vi "jymove.vi"() -> ()   [LabVIEW 2021]
uses:
  <vilib>/Math Plots/3D Math Plots/3D Scatter/3D Scatter XCtrl/3D Scatter.xctl
  <vilib>/Utility/file.llb/Write Delimited Spreadsheet (DBL).vi
  <vilib>/Math Plots/3D Math Plots/3D Scatter/3D Scatter Datatype/Public/Plot Helper (Matrix).vi
  <vilib>/Math Plots/3D Math Plots/3D Scatter/3D Scatter Datatype/3D Scatter Datatype.lvclass
  <vilib>/Analysis/NI_AALBase.lvlib
panel:
  out "Spectrum":cluster{"Y":dbl[], "Y":dbl[]}[](graph)
  out "波长数组 2":dbl[](array[numeric])
  out "data 2":i32[][](graph)
  out "Backlight":i32[][](graph)
  in  "选项卡控件":enum32{"IHR 550", "CCD", "MOVE"}(tab)
  out "Current UniqueID":string="Mono4"
  in  "Mono ID":string(combo)="Mono1"
  in  "Connect":bool
  out "Initialized JY":bool=TRUE
  in  "Force\nInitialization":bool
  in  "Target Grating":string(combo)="2"
  out "Current Description":string="1" caption="Description"
  out "Grating Index":i32=1
  out "Current Grating":dbl=1200.0
  out "Units":string="nm"
  out "Current WL":dbl=897.9988
  out "Exit Mirror\nPosition":i32(ring)=2 items=["EntranceMirror", "ExitMirror", "Front", "Side"]
  out "Entrance Mirror\nPosition":i32(ring)=2 items=["EntranceMirror", "ExitMirror", "Front", "Side"]
  out "Units 2":string="mm"
  out "Front Entrance":dbl
  in  "Target WL":dbl=710.0
  in  "Exit Mirror":u16(ring)=3 caption="Target Position Exit Mirror" items=["Front"=2, "Side"=3]
  in  "Entrance Mirror":u16(ring)=2 caption="Target Position\nEntrance Mirror" items=["Front"=2, "Side"=3]
  in  "Target\nFront Entrance":dbl=1.0
  in  "Move To\nTarget Positions":bool
  in  "initialize":bool
  in  "ShutterOpen":bool=TRUE caption="Shutter enable"
  in  "Acquire":bool
  in  "Temperature":bool
  in  "Setup":bool
  out "indicator":string="Ready !"
  in  "CCD Busy":bool
  in  "Continuous":bool
  out "initialized ?":bool=TRUE
  in  "Commande tab":T1(tab)
  in  "Area Number to Display":i32
  in  "Reformat":bool
  in  "GAIN":u16(ring)=2 caption="Device Name"
  in  "ADC":u16(ring) caption="Device Name"
  in  "Number of Areas :":u16=1 min=1 step=1
  in  "Integration time (ms) :":i16=2000
  out "Uniques ID":u16(ring)
  in  "Device Name":u16(ring)
  in  "Signal type :":enum16{"TTL Rising Edge", "TTL Falling Edge"}(ring)=enum."TTL Falling Edge"
  in  "Trigger Type :":u16(ring) items=["On Start"=1, "Per Acquisition"=2]
  in  "trigSigTypeString":string
  in  "trigEventString":string
  in  "Enable InputTriggers :":bool
  in  "Number of Cleans":i32=1
  in  "MultiAcqShutterMode":i32(ring)=3 items=["Open For All Spectra"=1, "Open for Each Spectrum"=3]
  in  "Accumulations:":u16=10 min=1 step=1
  in  "Multi Accumulation mode:":bool
  out "Y Pixels:":i32=256
  out "DataSize":i32=1024
  out "X Pixels:":i32=1024
  out "Firmware\nVersion":string="V1.20 CCD_4000"
  in  "Save Backlight":bool
  in  "起始波长":dbl=693.352
  in  "终止波长":dbl=726.407
  in  "扫描方式":enum32{"起始扫描", "半径扫描"}(tab)
  in  "y轴起始位置":sgl=5.355 min=-150 max=150 format="%#.6g"
  in  "y轴步进长度":sgl=0.0008 min=-150 max=150 format="%.4g"
  in  "y轴终止位置":sgl=5.359 min=-150 max=150 format="%#.6g"
  in  "x轴起始位置":dbl=5.495
  in  "x轴步进长度":dbl=0.0008
  in  "x轴终止位置":dbl=5.535
  in  "中心X":dbl=10.0
  in  "中心Y":dbl=10.0
  in  "X步长":dbl=0.5
  in  "Y半径":dbl=5.0
  in  "X半径":dbl=5.0
  in  "Y步长":dbl=0.5
  in  "x 位置":dbl=5.495
  in  "y 位置":sgl=5.35 min=-150 max=150 format="%#.6g"
  in  "移动":bool
  out "Acq Time(ms)":u32=3401
  out "位置":dbl[](array[numeric]) format="%.10e"
  in  "开始采集":bool
  out "采集进度":u8(slide) scale=0.0..100.0
  out "最终存储路径":path
  out "Intensity":dbl
  out "POINT":dbl
  out "JYCCDLib.IJYCCDReqd":refnum<k7>
  in  "计数器":dbl=720.0
  out "error out":errorcluster
  out "Gratings":dbl[](array[numeric])=[1200.0, 300.0]
  out "Data":i32[][](graph)
  out "trigAddress":i32
  out "Gain Number":i32[](array[numeric])=[10, 11, 12, 13, 8, 2]
  out "ADC Number":i32[](array[numeric])=[0, 1, 2, 3, 4]
  out "temp graph":dbl(graph)=-134.538067
  in  "Close":bool=TRUE
  out "areas :":i32[][](array[numeric])=[[1], [1], [1], [1024], [256], [1], [256]]
  in  "Constante de condition\n(Voir l'aide contextuelle)":bool
  out "波长3维图":refnum<class "3D Plot Datatype.lvclass">[](xcontrol)
  out "强度三维图":refnum<class "3D Plot Datatype.lvclass">[](xcontrol)
  out "起始位置":dbl[](array[numeric])
  in  "x":dbl=10.0
  in  "y":sgl=1.0 min=-150 max=150 format="%#.6g"
  out "强度数组":dbl[][](array[numeric])
  out "波长数组":dbl[][](array[numeric])
  out "X循环次数":dbl
  out "Y循环次数":sgl
  in  "Y移动量":dbl[](array[numeric]) format="%.6f"
  in  "X移动量":dbl[](array[numeric]) format="%.6f"
  in  "Group Name (250 c max)":string="XY"
  in  "PASSWORD":string="Administrator"
  in  "USER NAME":string="Administrator"
  in  "IP Address":string="192.168.0.254"
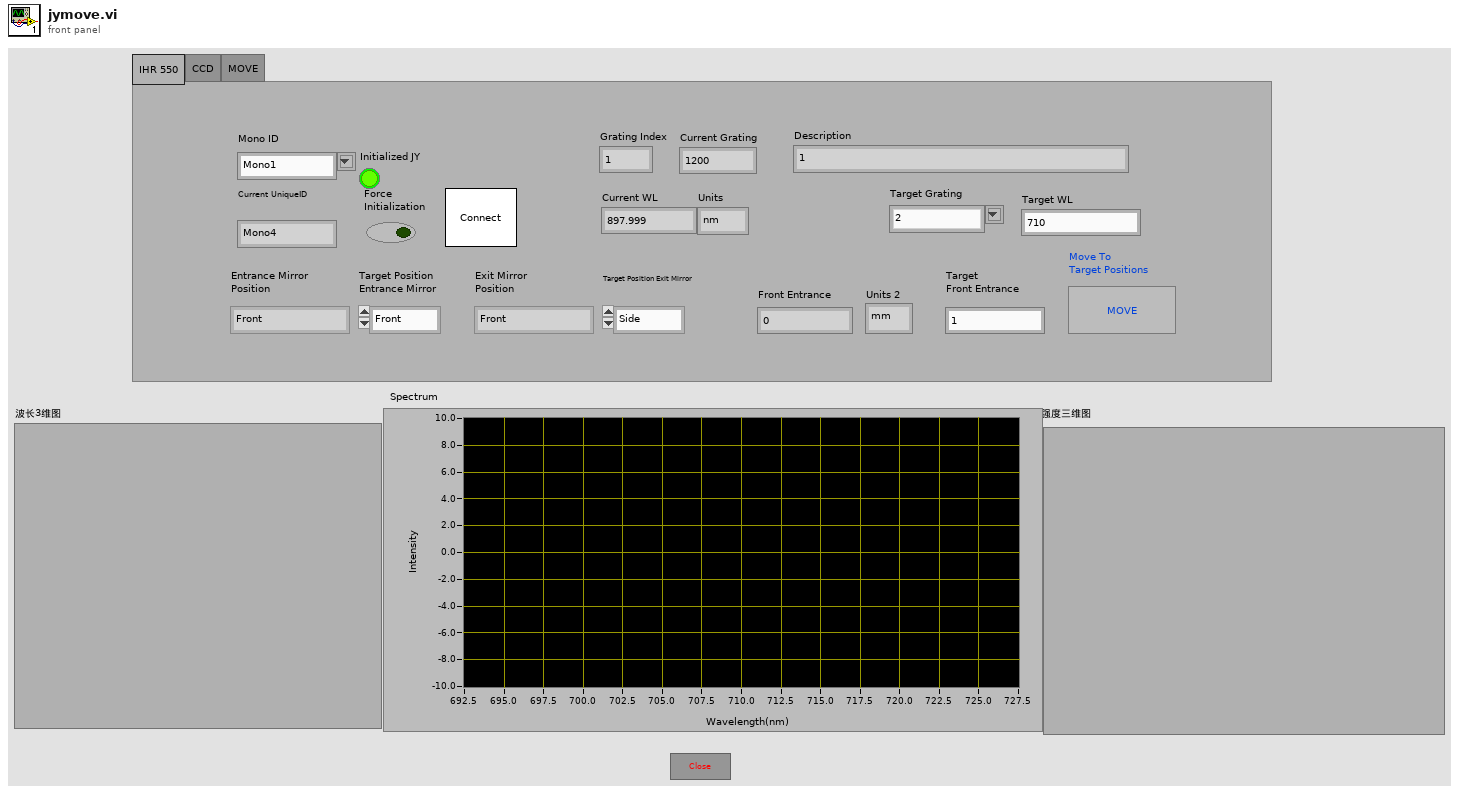
[diagram p1: front panel]
types:
  T1 = enum32{"Settings", "Trigger In", "Multi-Accu.", "Infos"}
  T2 = cluster{"connection TCP":refnum<k5>, "LogTo File":bool, "Log File refnum":refnum<file>, "no error if error log":bool}
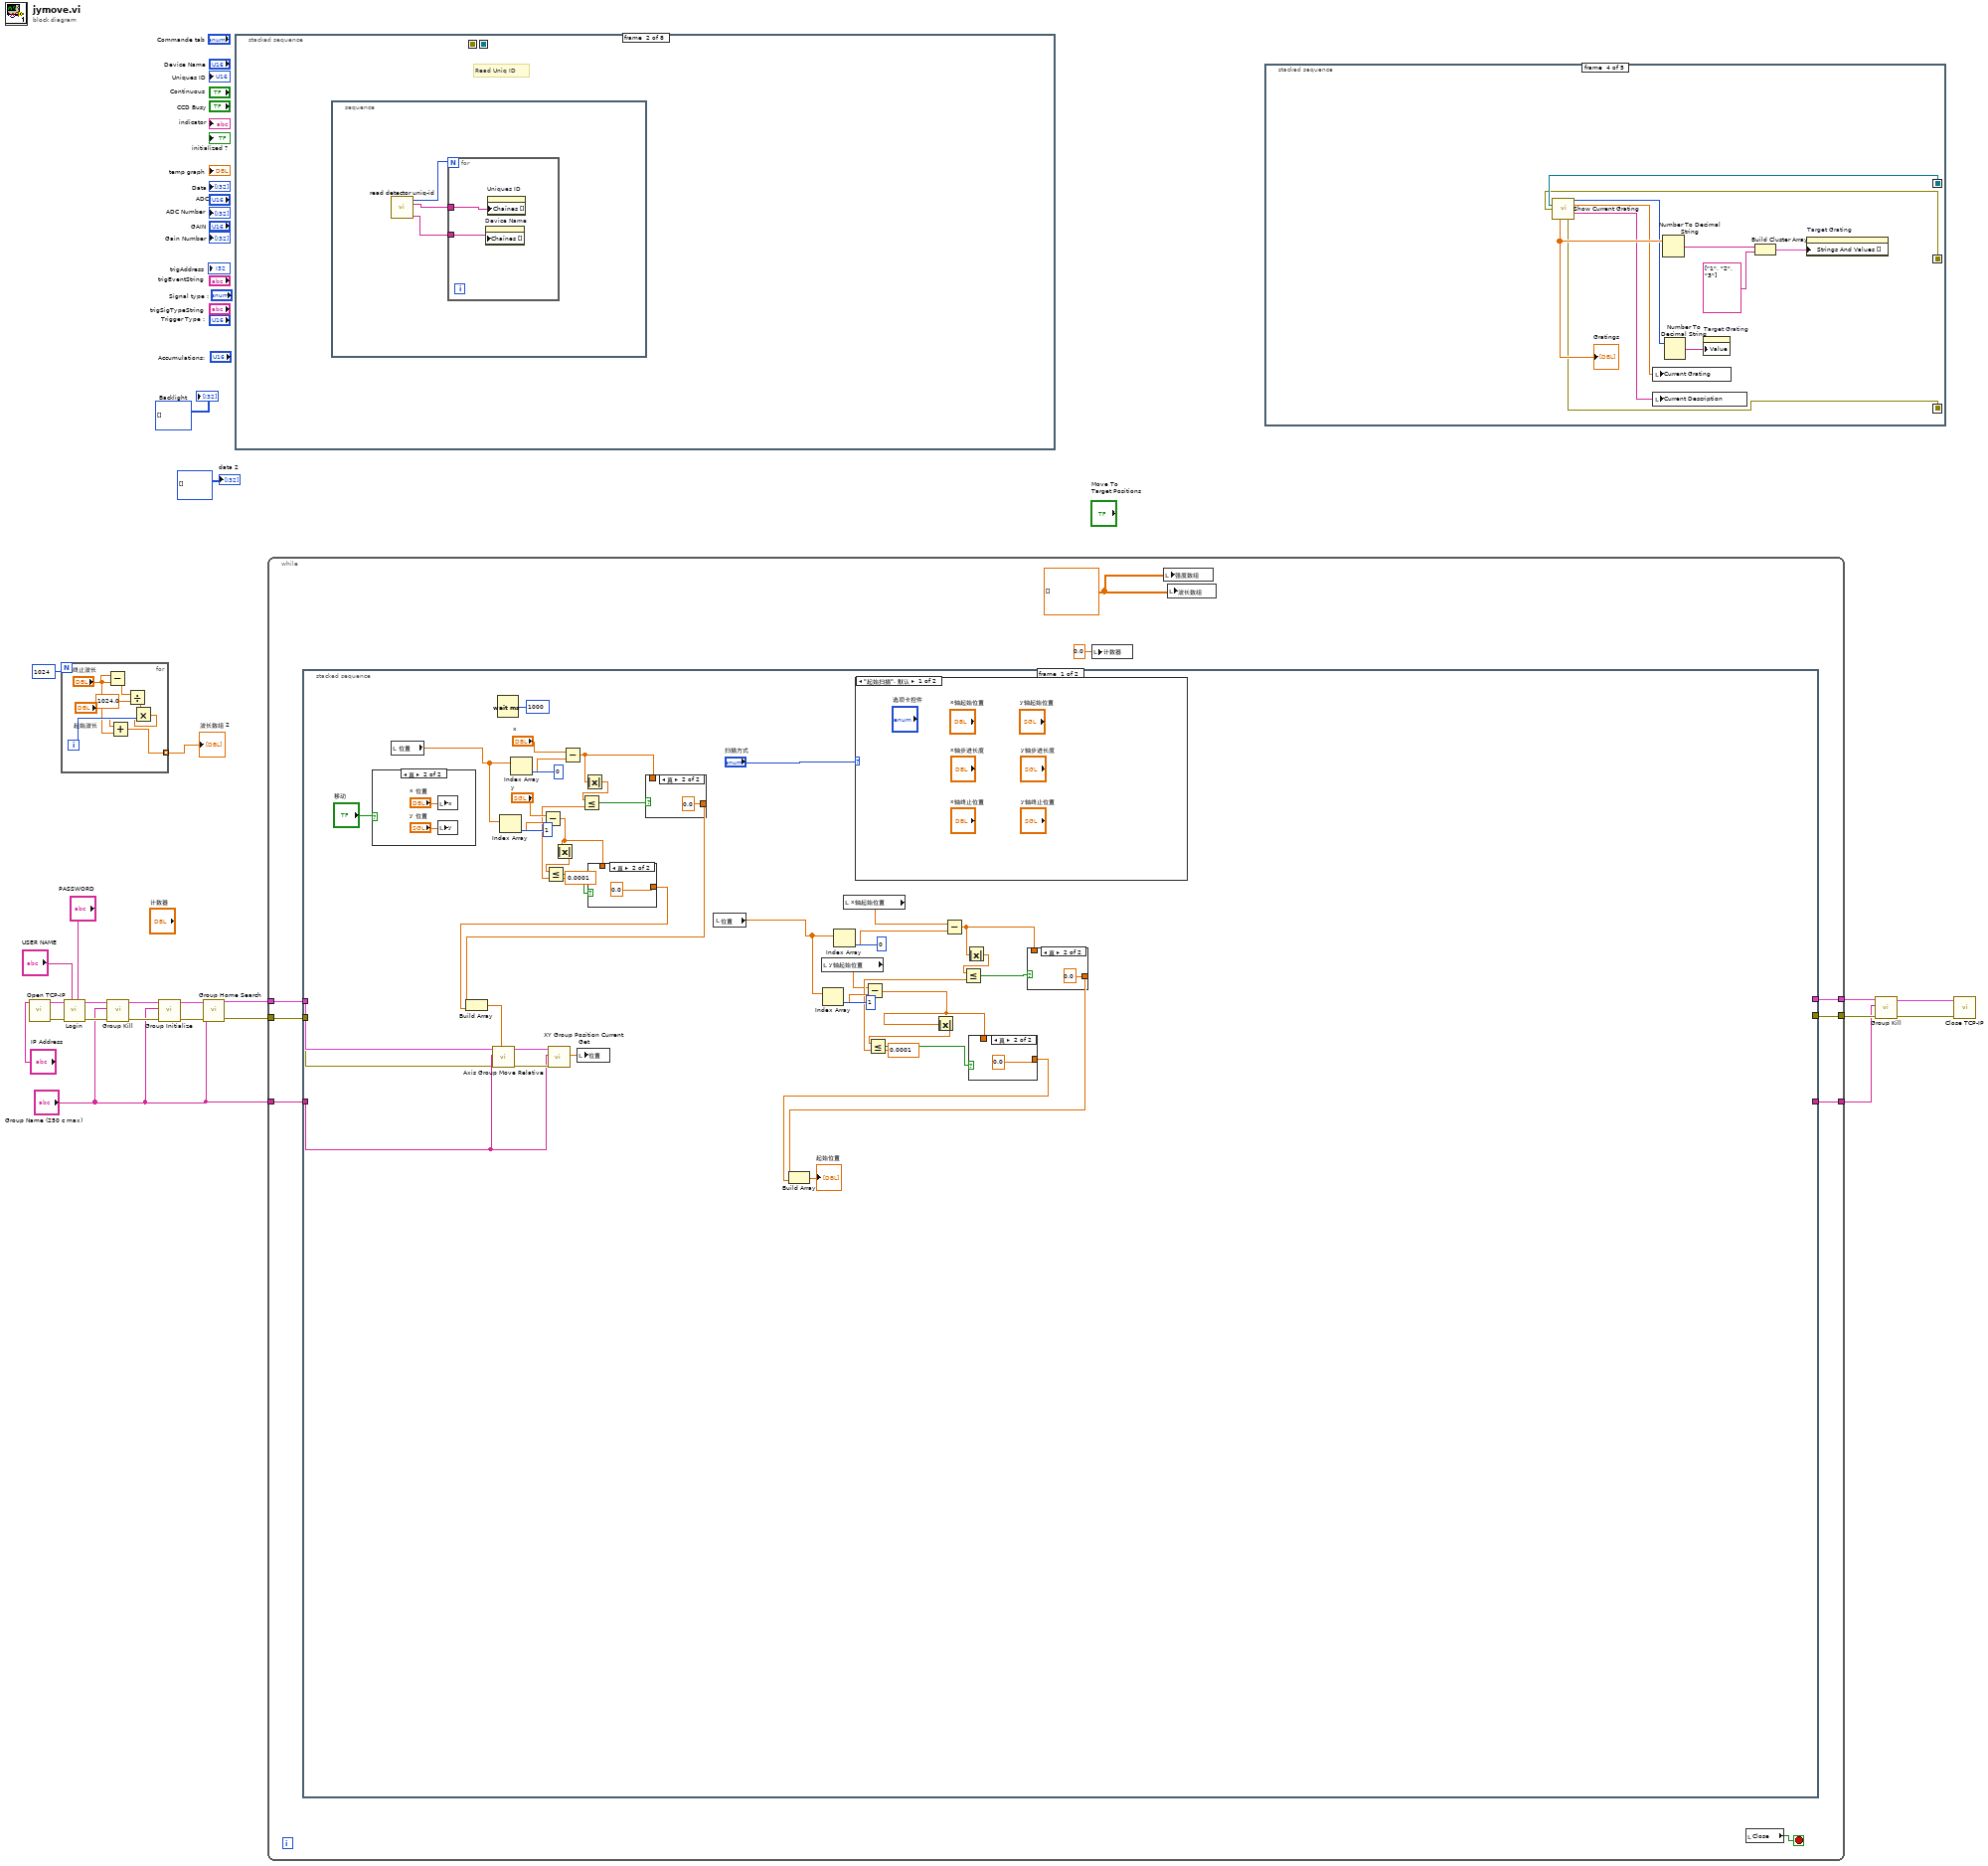
[diagram p0: block diagram]
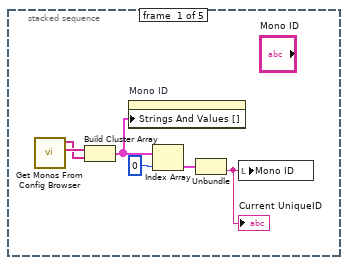
[diagram p2: hidden frame]
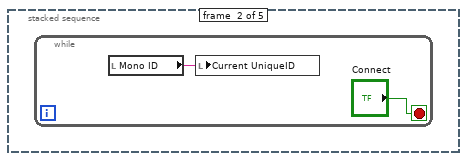
[diagram p3: hidden frame]
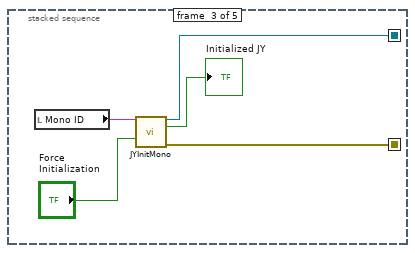
[diagram p4: hidden frame]
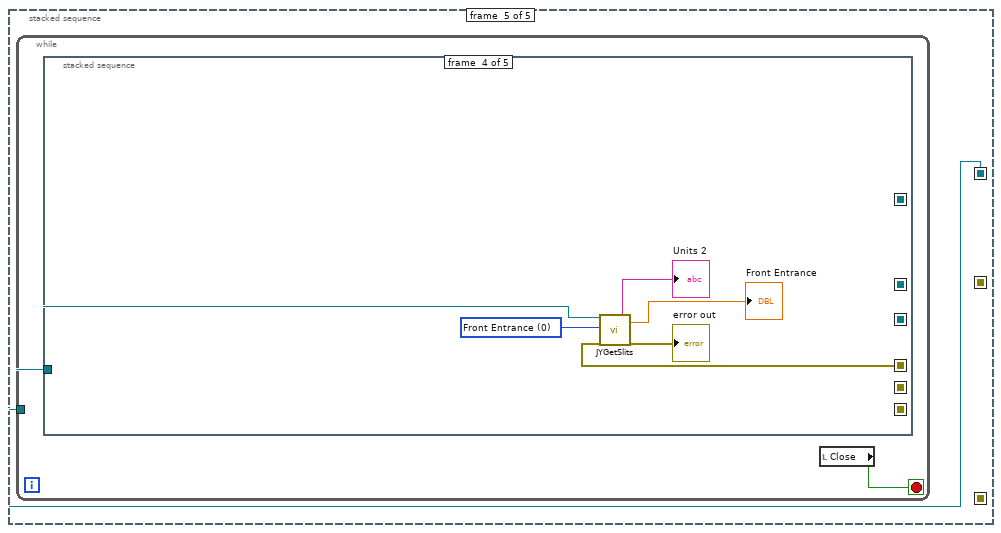
[diagram p5: hidden frame]
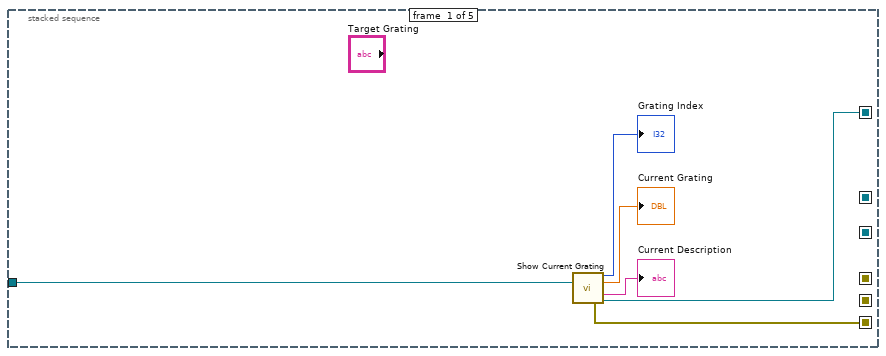
[diagram p6: hidden frame]
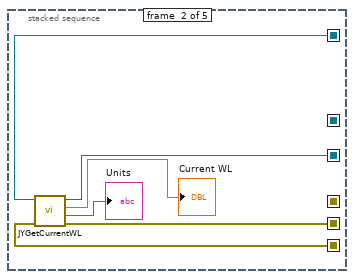
[diagram p7: hidden frame]
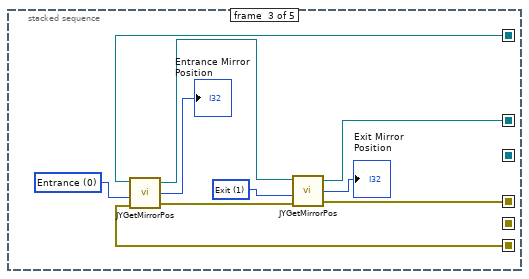
[diagram p8: hidden frame]
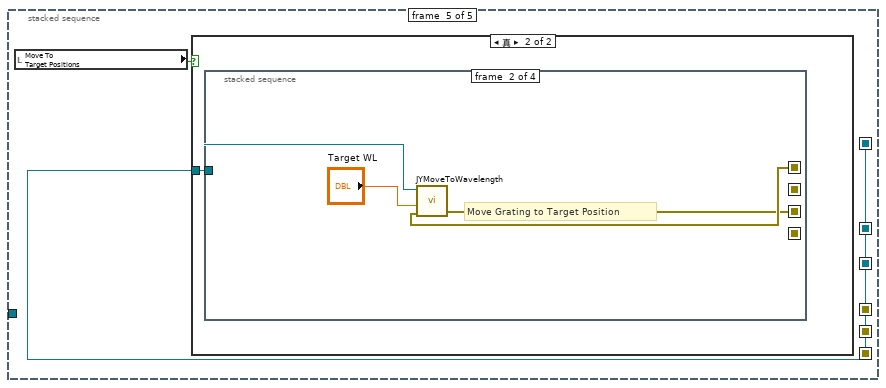
[diagram p9: hidden frame]
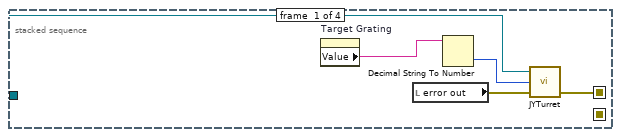
[diagram p11: hidden frame]
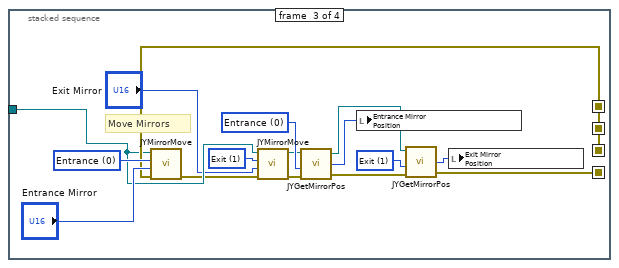
[diagram p12: hidden frame]
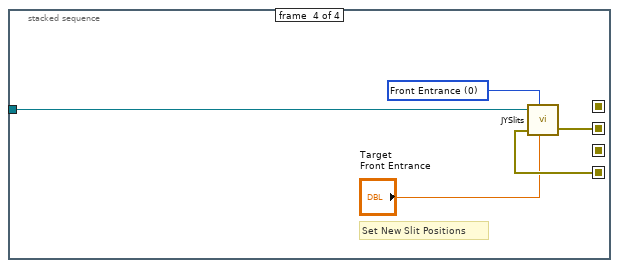
[diagram p13: hidden frame]
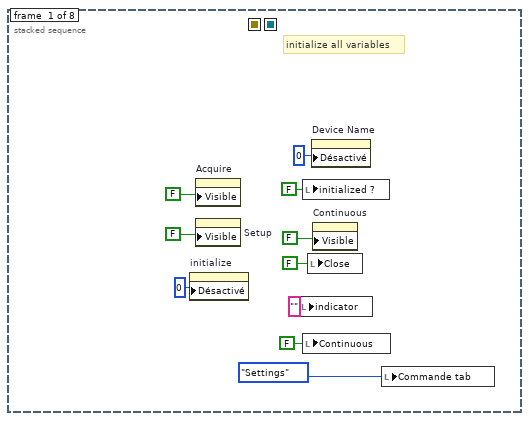
[diagram p14: hidden frame]
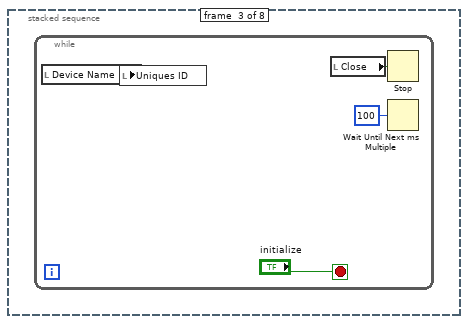
[diagram p15: hidden frame]
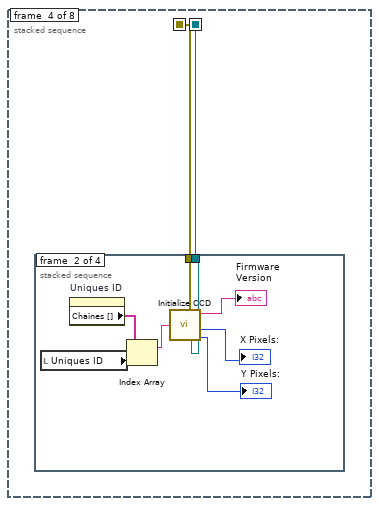
[diagram p16: hidden frame]
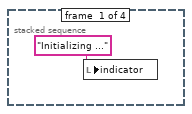
[diagram p17: hidden frame]
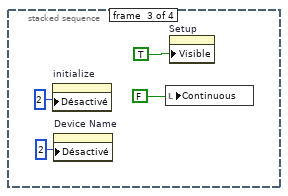
[diagram p18: hidden frame]
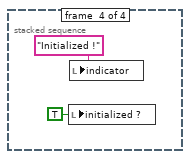
[diagram p19: hidden frame]
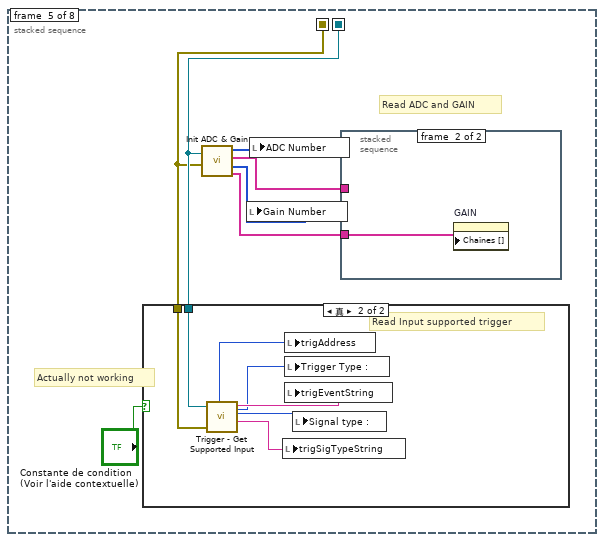
[diagram p20: hidden frame]
diagram:
  n1 = call "Open TCP-IP.vi"("IP address"="IP Address") -> ("error out"=w23:errorcluster, "Connection ID"=w22:T2)  [unwired: 8 in, 1 out]
  n2 = for {
    N: 1024 -> [_]
    tunnel: [w28] -> w1 mode=indexing
    i -> [w30]
    n3 = Subtract(x="终止波长", y="起始波长") -> (x-y=w26:dbl)
    n4 = Divide(x=w26, y=1024.0) -> (x/y=w24:dbl)
    n5 = Multiply(x=w24, y=w30) -> (x*y=w29:dbl)
    n6 = Add(x=w29, y="起始波长") -> (x+y=w28:dbl)
  }
  "波长数组 2" <- w1
  n7 = call "Login.vi"("Password"="PASSWORD", "User"="USER NAME", "error in (no error)"=w23, "connection ID in"=w22) -> ("error out"=w15:errorcluster, "connection ID out"=w16:T2)  [unwired: 5 in, 1 out]
  n8 = call "Group Kill.vi"("error in (no error)"=w15, "Group Name (250 c max)"="Group Name (250 c max)", "connection ID in"=w16) -> ("error out"=w17:errorcluster, "connection ID out"=w18:T2)  [unwired: 6 in, 1 out]
  n9 = call "Group Initialize.vi"("error in (no error)"=w17, "Group Name (250 c max)"="Group Name (250 c max)", "connection ID in"=w18) -> ("error out"=w13:errorcluster, "connection ID out"=w14:T2)  [unwired: 6 in, 1 out]
  n10 = call "Group Home Search.vi"("error in (no error)"=w13, "Group Name (250 c max)"="Group Name (250 c max)", "connection ID in"=w14) -> ("error out"=w11:errorcluster, "connection ID out"=w12:T2)  [unwired: 6 in, 1 out]
  n11 = stacked-sequence {
    seq-local: [_ _ _ w52 _ _ _ _] -> [_ _ _ _ w70 w90 w93 w191]
    seq-local: [_ _ _ w51 _ _ _ _] -> [_ _ _ _ w71 w91 w92 w192]
    frame #0 {
      # "initialize all variables"
      n12 = property on="initialize" class="Bool"("Désactivé"=u8 0) -> ()  [unwired: 2 in, 2 out]
      n13 = property on="Acquire" class="Bool"("Visible"=FALSE) -> ()  [unwired: 2 in, 2 out]
      n14 = property on="Setup" class="Bool"("Visible"=FALSE) -> ()  [unwired: 2 in, 2 out]
      n15 = local write "indicator"("" ("indicator")) -> ()
      n16 = local write "initialized ?"(FALSE ("initialized ?")) -> ()
      n17 = local write "Continuous"(FALSE ("Continuous")) -> ()
      n18 = local write "Close"(FALSE ("Close")) -> ()
      n19 = property on="Device Name" class="Ring (严格)"("Désactivé"=u8 0) -> ()  [unwired: 2 in, 2 out]
      n20 = property on="Continuous" class="Bool (严格)"("Visible"=FALSE) -> ()  [unwired: 2 in, 2 out]
      n21 = local write "Commande tab"(T1."Settings" ("Commande tab")) -> ()
    }
    frame #1 {
      # "Read Uniq ID"
      n22 = stacked-sequence {
        frame #0 {
          n23 = call "read detector uniq-id.vi"() -> ("nbr of components"=w44:i32, "UniqueID"=w43:string[], "Name"=w42:string[])  [unwired: 4 out]
          n24 = for {
            N: w44 -> [_]
            tunnel: w43 -> [w46]
            tunnel: w42 -> [w45]
            n25 = property on="Device Name" class="Ring (严格)"("Chaînes []"=w45) -> ()  [unwired: 2 in, 2 out]
            n26 = property on="Uniques ID" class="Ring (严格)"("Chaînes []"=w46) -> ()  [unwired: 2 in, 2 out]
          }
        }
      }
    }
    frame #2 {
      n27 = while {
        stop <- "initialize" stop-if-true
        n28 = local read "Device Name"() -> (w49:u16)
        n29 = local write "Uniques ID"(w49) -> ()
        n30 = local read "Close"() -> (w47:bool)
        n31 = Stop(stop? (T)=w47) -> ()
        n32 = Wait Until Next ms Multiple(millisecond multiple=u32 100 ("n millisecondes")) -> ()  [unwired: 1 out]
      }
    }
    frame #3 {
      n33 = stacked-sequence {
        tunnel: [_ w59 _ _] -> w52
        tunnel: [_ w58 _ _] -> w51
        frame #0 {
          n34 = local write "indicator"("Initializing ..." ("indicator")) -> ()
        }
        frame #1 {
          n35 = local read "Uniques ID"() -> (w56:u16)
          n36 = property on="Uniques ID" class="Ring (严格)"() -> ("Chaînes []"=w57:string[])  [unwired: 2 in, 2 out]
          n37 = Index Array(array=w57, index=w56) -> (element=w55:string)
          n38 = call "Initialize CCD.vi"("Unique id:"=w55) -> ("activeYPixels"=→"Y Pixels:":i32, "JYCCDLib.IJYCCDReqd"=w58:refnum<k7>, "activeXPixels"=→"X Pixels:":i32, "sortie d'erreur"=w59:errorcluster, "FirmwareVersion"=→"Firmware\nVersion":string)  [unwired: 3 out]
        }
        frame #2 {
          n39 = property on="initialize" class="Bool"("Désactivé"=u8 2) -> ()  [unwired: 2 in, 2 out]
          n40 = property on="Device Name" class="Ring (严格)"("Désactivé"=u8 2) -> ()  [unwired: 2 in, 2 out]
          n41 = local write "Continuous"(FALSE ("Continuous")) -> ()
          n42 = property on="Setup" class="Bool"("Visible"=TRUE) -> ()  [unwired: 2 in, 2 out]
        }
        frame #3 {
          n43 = local write "initialized ?"(TRUE ("initialized ?")) -> ()
          n44 = local write "indicator"("Initialized !" ("indicator")) -> ()
        }
      }
    }
    frame #4 {
      # "Actually not working"
      # "Read ADC and GAIN"
      n45 = case shown="真" "Constante de condition\n(Voir l'aide contextuelle)" {
        tunnel: w71 -> [_ w81]
        tunnel: w70 -> [_ w80]
        frame False {
        }
        frame True {
          # "Read Input supported trigger"
          n46 = call "Trigger - Get Supported Input.vi"("JYCCDLib.IJYCCDReqd"=w81, "Error Input"=w80) -> ("trigAddress"=w75:i32, "eventPtr"=w76:i32, "trigEventString"=w79:string, "trigSigType"=w78:i32, "trigSigTypeString"=w77:string)  [unwired: 4 out]
          n47 = local write "trigSigTypeString"(w77) -> ()
          n48 = local write "trigAddress"(w75) -> ()
          n49 = local write "Trigger Type :"(w76) -> ()
          n50 = local write "trigEventString"(w79) -> ()
          n51 = local write "Signal type :"(w78) -> ()
        }
      }
      n52 = call "Init ADC & Gain.vi"("JYCCDLib.IJYCCDReqd"=w71, "input error"=w70) -> ("ADC Number"=w69:i32[], "ADC description"=w74:string[], "Gain Number"=w72:i32[], "Gain description"=w73:string[])
      n53 = local write "Gain Number"(w72) -> ()
      n54 = local write "ADC Number"(w69) -> ()
      n55 = stacked-sequence {
        tunnel: w74 -> [w82 _]
        tunnel: w73 -> [_ w83]
        frame #0 {
          n56 = property on="ADC" class="Ring (严格)"("Chaînes []"=w82) -> ()  [unwired: 2 in, 2 out]
        }
        frame #1 {
          n57 = property on="GAIN" class="Ring (严格)"("Chaînes []"=w83) -> ()  [unwired: 2 in, 2 out]
        }
      }
    }
    frame #5 {
      # "IS multi Accumulation Supported ?"
      n58 = call "MultiAccu - Is Supported.vi"("Error In"=w90, "JYCCDLib.IJYCCDReqd"=w91) -> ("IsOperatingModeSupported"=w84:bool)  [unwired: 3 out]
      n59 = Select(t=0, s=w84, f=2) -> (s? t:f=w87:i32)
      n60 = Select(t=FALSE, s=w84, f=w84) -> (s? t:f=w86:bool)
      n61 = local write "Multi Accumulation mode:"(w86) -> ()
      n62 = property on="Multi Accumulation mode:" class="Bool (严格)"("Désactivé"=w87) -> ()  [unwired: 2 in, 2 out]
      n63 = property on="Multi Accumulation mode:" class="Bool (严格)"("Désactivé"=w87) -> ()  [unwired: 2 in, 2 out]
    }
    frame #6 {
      n64 = while {
        tunnel: w92 -> [w100]
        tunnel: w93 -> [w99]
        stop <- "Close" stop-if-true
        n65 = case shown="真" "Reformat" {
          frame False {
          }
          frame True {
            n66 = local read "Y Pixels:"() -> (w169:i32)
            n67 = local read "X Pixels:"() -> (w171:i32)
            n68 = call "Spectral Reformat CCD area.vi"("Y Pixels:"=w169, "X Pixels:"=w171, "numAreas"="Number of Areas :") -> ("areas :"=→"areas :":i32[][])  [unwired: 3 out]
          }
        }
        n69 = case shown="真" "Setup" {
          tunnel: w99 -> [_ w174]
          tunnel: w100 -> [_ w173]
          frame False {
          }
          frame True {
            n70 = stacked-sequence {
              tunnel: w174 -> [_ w188 _]
              tunnel: w173 -> [_ w176 _]
              frame #0 {
                n71 = local write "indicator"("Setting up the detector" ("indicator")) -> ()
              }
              frame #1 {
                w186 = 1 items=["JYMCD_ACQ_FORMAT_IMAGE", "JYMCD_ACQ_FORMAT_SCAN"] ("Acquisition type")
                n72 = local read "Gain Number"() -> (w181:i32[])
                n73 = local read "GAIN"() -> (w177:u16)
                n74 = local read "ADC Number"() -> (w182:i32[])
                n75 = local read "ADC"() -> (w178:u16)
                n76 = Index Array(array=w181, index=w177) -> (element=w179:i32)
                n77 = Index Array(array=w182, index=w178) -> (element=w180:i32)
                n78 = local read "Number of Areas :"() -> (w184:u16)
                n79 = local read "areas :"() -> (w185:i32[][])
                n80 = call "Setup CCD.vi"("numAreas"=w184, "areas :"=w185, "JYCCDLib.IJYCCDReqd"=w176, "entrée d'erreur (pas d'erreur)"=w188, "Acquisition type"=w186, "Gain"=w179, "Select ADC"=w180, "Integration time(ms)"="Integration time (ms) :") -> ("DataSize"=→"DataSize":i32)  [unwired: 1 out]
                "JYCCDLib.IJYCCDReqd" <- w176
              }
              frame #2 {
                w189 = TRUE ("Visible")
                n81 = property on="Continuous" class="Bool (严格)"("Visible"=w189) -> ()  [unwired: 2 in, 2 out]
                n82 = property on="Acquire" class="Bool"("Visible"=w189) -> ()  [unwired: 2 in, 2 out]
                n83 = local write "indicator"("Ready !" ("indicator")) -> ()
              }
            }
          }
        }
        n84 = local read "Accumulations:"() -> (w96:u16)
        n85 = local read "Continuous"() -> (w101:bool)
        n86 = Or(x="Acquire", y=w101) -> (x .or. y?=w98:bool)
        n87 = case shown="真" w98 {
          tunnel: w100 -> [_ w113]
          tunnel: w99 -> [_ w112]
          tunnel: "Enable InputTriggers :" -> [_ w111]
          tunnel: "Multi Accumulation mode:" -> [_ w110]
          tunnel: w96 -> [_ w109]
          tunnel: "MultiAcqShutterMode" -> [_ w108]
          frame False {
          }
          frame True {
            n88 = stacked-sequence {
              seq-local: [_ _ w126 _ _] -> [_ _ _ w154 _]
              tunnel: w113 -> [_ w115 w130 w153 _]
              tunnel: w112 -> [_ w116 w129 w152 _]
              tunnel: w111 -> [_ w117 _ _ _]
              tunnel: w110 -> [_ _ w128 _ _]
              tunnel: w109 -> [_ _ w127 _ _]
              tunnel: w108 -> [_ _ w125 _ _]
              frame #0 {
                n89 = local write "CCD Busy"(TRUE ("CCD Busy")) -> ()
              }
              frame #1 {
                n90 = case shown="真" w117 {
                  tunnel: w116 -> [w118 w124]
                  tunnel: w115 -> [w119 w123]
                  frame False {
                    n91 = call "Trigger - Disable.vi"("Error In"=w118, "JYCCDLib.IJYCCDReqd"=w119) -> ()  [unwired: 6 out]
                  }
                  frame True {
                    n92 = local read "Trigger Type :"() -> (w120:u16)
                    n93 = local read "Signal type :"() -> (w121:enum16{"TTL Rising Edge", "TTL Falling Edge"})
                    n94 = local read "trigAddress"() -> (w122:i32)
                    n95 = call "Trigger - Enable.vi"("Error In"=w124, "sigType"=w121, "event"=w120, "trigAddress"=w122, "JYCCDLib.IJYCCDReqd"=w123) -> ()  [unwired: 3 out]
                  }
                }
              }
              frame #2 {
                n96 = case shown="真" w128 {
                  selector: w128 -> [_ w136]
                  tunnel: w130 -> [w133 w139]
                  tunnel: w129 -> [w132 w138]
                  tunnel: w127 -> [_ w137]
                  tunnel: [u16 1 ("Accumulations:") w137] -> w126
                  tunnel: w125 -> [_ w135]
                  frame False {
                    n97 = call "MultiAccu - Disable.vi"("Error In"=w132, "JYCCDLib.IJYCCDReqd"=w133) -> ()  [unwired: 4 out]
                  }
                  frame True {
                    n98 = call "MultiAccu - Configure.vi"("JYCCDLib.IJYCCDReqd"=w139, "Cleans Before"="Number of Cleans", "Accumulations:"=w137, "MultiAcqHardwareMode"=w136, "MultiAcqShutterMode"=w135, "Error In"=w138) -> ()  [unwired: 1 in, 9 out]
                  }
                }
              }
              frame #3 {
                n99 = call "MultiAccu - Acquire spectral.vi"("error in"=w152, "Accumulations:"=w154, "ShutterOpen"="ShutterOpen", "JYCCDLib.IJYCCDReqd"=w153) -> ("Acq Time(ms)"=→"Acq Time(ms)":u32, "Array Out"=w151:i32[][][])  [unwired: 1 out]
                n100 = call "Array reset dimension.vi"("Area Number"="Area Number to Display", "Array In"=w151) -> ("Array Out"=w149:i32[][])
                n101 = local read "Backlight"() -> (w148:i32[][])
                n102 = Subtract(x=w149, y=w148) -> (x-y=w145:i32[][])
                n103 = local write "Data"(w149) -> ()
                n104 = local write "data 2"(w145) -> ()
                n105 = Index Array(array=w145, index (row)=0 ("禁用的索引 (列)")) -> (element=w146:i32[])  [unwired: 1 in]
                n106 = local read "波长数组 2"() -> (w142:dbl[])
                n107 = Reverse 1D Array(array=w146) -> (reversed array=w144:i32[])
                n108 = call "转换至动态数据2"("Array"=w142) -> ("Dynamic Data Type"=w141:dynamicdata)  [unwired: 3 in]
                n109 = call "转换至动态数据"("Array"=w144) -> ("Dynamic Data Type"=w143:dynamicdata)  [unwired: 3 in]
                n110 = call "Build XY Graph2"("Y Input"=w143, "X Input"=w141) -> ("XY Graph"=w140:cluster{"Y":dbl[], "Y":dbl[]}[])  [unwired: 8 in, 1 out]
                n111 = local write "Spectrum"(w140) -> ()
              }
              frame #4 {
                n112 = case shown="真" "Save Backlight" {
                  frame False {
                  }
                  frame True {
                    n113 = local read "Data"() -> (w160:i32[][])
                    n114 = local write "Backlight"(w160) -> ()
                    n115 = local write "Save Backlight"(FALSE ("Save Backlight")) -> ()
                  }
                }
                n116 = local write "CCD Busy"(FALSE ("CCD Busy")) -> ()
              }
            }
          }
        }
        n117 = case shown="真" "Temperature" {
          tunnel: w100 -> [_ w163]
          tunnel: w99 -> [_ w162]
          frame False {
            n118 = property on="temp graph" class="WFChart (严格)"("Visible"=FALSE) -> ()  [unwired: 2 in, 2 out]
          }
          frame True {
            n119 = stacked-sequence {
              tunnel: w163 -> [_ w168]
              tunnel: w162 -> [_ w167]
              frame #0 {
                n120 = property on="temp graph" class="WFChart (严格)"("Visible"=TRUE) -> ()  [unwired: 2 in, 2 out]
              }
              frame #1 {
                w166 = u16 0 items=["° Celsius", "Kelvin", "° Farenheit"] ("units")
                n121 = call "read temperature.vi"("entrée d'erreur (pas d'erreur)"=w167, "units"=w166, "JYCCDLib.IJYCCDReqd"=w168) -> ("Current Temperature"=w165:dbl)
                n122 = local write "temp graph"(w165) -> ()
              }
            }
          }
        }
        n123 = Wait Until Next ms Multiple(millisecond multiple=u32 50 ("n millisecondes")) -> ()  [unwired: 1 out]
      }
    }
    frame #7 {
      n124 = Close Reference(reference=w192, error in (no error)=w191) -> ()  [unwired: 1 out]
    }
  }
  n125 = while {
    tunnel: w12 -> [w200]
    tunnel: w11 -> [w199]
    tunnel: "Group Name (250 c max)" -> [w198]
    tunnel: [w197] -> w7
    tunnel: [w196] -> w6
    tunnel: [w195] -> w5
    stop <- w193 stop-if-true
    w201 = dbl[][] [] ("Spectral Array")
    n126 = stacked-sequence {
      tunnel: w200 -> [w223 w270]
      tunnel: w199 -> [w222 w269]
      tunnel: w198 -> [w224 w268]
      tunnel: [_ w267] -> w197
      tunnel: [_ w266] -> w196
      tunnel: [_ w265] -> w195
      frame #0 {
        w212 = 0.0001 ("y")
        w233 = 0.0001 ("y")
        n127 = case shown="真" "移动" {
          frame False {
          }
          frame True {
            n128 = local write "x"("x 位置") -> ()
            n129 = local write "y"("y 位置") -> ()
          }
        }
        n130 = local read "位置"() -> (w242:dbl[])
        n131 = Wait (ms)(milliseconds to wait=u32 1000 ("等待时间（毫秒）")) -> ()  [unwired: 1 out]
        n132 = Index Array(array=w242, index=1 ("索引")) -> (element=w237:dbl)
        n133 = Index Array(array=w242, index=0 ("索引")) -> (element=w239:dbl)
        n134 = Subtract(x="y", y=w237) -> (x-y=w234:dbl)
        n135 = Absolute Value(x=w234) -> (abs(x)=w228:dbl)
        n136 = Less Or Equal?(x=w228, y=w233) -> (x <= y?=w229:bool)
        n137 = Subtract(x="x", y=w239) -> (x-y=w232:dbl)
        n138 = Absolute Value(x=w232) -> (abs(x)=w227:dbl)
        n139 = Less Or Equal?(x=w227, y=w233) -> (x <= y?=w230:bool)
        n140 = case shown="真" w229 {
          tunnel: [w253 0.0] -> w235
          tunnel: w234 -> [w253 _]
          frame False {
          }
          frame True {
          }
        }
        n141 = case shown="真" w230 {
          tunnel: w232 -> [w251 _]
          tunnel: [w251 0.0] -> w231
          frame False {
          }
          frame True {
          }
        }
        n142 = Build Array(w231, w235) -> (w221:dbl[])
        n143 = call "Axis Group Move Relative.vi"("Target Displacement (units)"=w221, "error in (no error)"=w222, "Group Name (250 c max)"=w224, "connection ID in"=w223) -> ("error out"=w225:errorcluster, "connection ID out"=w226:T2)  [unwired: 5 in, 1 out]
        n144 = call "XY Group Position Current Get.vi"("error in (no error)"=w225, "XY Group Name (250 c max)"=w224, "connection ID in"=w226) -> ("Current Position X & Y (units)"=w220:dbl[])  [unwired: 5 in, 3 out]
        n145 = local write "位置"(w220) -> ()
        n146 = local read "位置"() -> (w218:dbl[])
        n147 = local read "y轴起始位置"() -> (w204:sgl)
        n148 = Index Array(array=w218, index=1 ("索引")) -> (element=w215:dbl)
        n149 = Index Array(array=w218, index=0 ("索引")) -> (element=w216:dbl)
        n150 = local read "x轴起始位置"() -> (w205:dbl)
        n151 = case shown="\"起始扫描\", 默认" "扫描方式" {
          frame "起始扫描", Default {
          }
          frame "半径扫描" {
            n152 = local write "x轴步进长度"("X步长") -> ()
            n153 = Add(x="X半径", y="中心X") -> (x+y=w264:dbl)
            n154 = Subtract(x="中心X", y="X半径") -> (x-y=w261:dbl)
            n155 = local write "x轴终止位置"(w264) -> ()
            n156 = local write "x轴起始位置"(w261) -> ()
            n157 = Add(x="Y半径", y="中心Y") -> (x+y=w256:dbl)
            n158 = Subtract(x="中心Y", y="Y半径") -> (x-y=w257:dbl)
            n159 = local write "y轴步进长度"("Y步长") -> ()
            n160 = local write "y轴终止位置"(w256) -> ()
            n161 = local write "y轴起始位置"(w257) -> ()
          }
        }
        n162 = Subtract(x=w204, y=w215) -> (x-y=w213:dbl)
        n163 = Absolute Value(x=w213) -> (abs(x)=w207:dbl)
        n164 = Less Or Equal?(x=w207, y=w212) -> (x <= y?=w208:bool)
        n165 = Subtract(x=w205, y=w216) -> (x-y=w211:dbl)
        n166 = Absolute Value(x=w211) -> (abs(x)=w206:dbl)
        n167 = Less Or Equal?(x=w206, y=w212) -> (x <= y?=w209:bool)
        n168 = case shown="真" w208 {
          tunnel: [w249 0.0] -> w214
          tunnel: w213 -> [w249 _]
          frame False {
          }
          frame True {
          }
        }
        n169 = case shown="真" w209 {
          tunnel: w211 -> [w247 _]
          tunnel: [w247 0.0] -> w210
          frame False {
          }
          frame True {
          }
        }
        n170 = Build Array(w210, w214) -> (→"起始位置":dbl[])
      }
      frame #1 {
        n171 = case shown="真" "开始采集" {
          tunnel: w270 -> [w274 w318]
          tunnel: w268 -> [w272 w316]
          tunnel: w269 -> [w273 w317]
          tunnel: [w274 w300] -> w267
          tunnel: [w273 w299] -> w266
          tunnel: [w272 w298] -> w265
          frame False {
            n172 = stacked-sequence {
              frame #0 {
                n173 = Current VI's Path() -> (path=w291:path)
                n174 = Get Date/Time In Seconds() -> (seconds since 1Jan1904=w288:timestamp)
                n175 = Strip Path(path=w291) -> (stripped path=w290:path)  [unwired: 1 out]
                n176 = Path To String(path=w290) -> (string=w287:string)
                n177 = Format Date/Time String(time format string (%c)="%m.%d" ("时间格式字符串(%c)"), seconds (now)=w288) -> (date/time string=w280:string)  [unwired: 1 in]
                n178 = Concatenate Strings(w287, "\\Save\\" ("字符串"), w280) -> (w285:string)
                n179 = String To Path(string=w285) -> (path=w284:path)
                n180 = call <vilib>:"Check if File or Folder Exists.vi"("path"=w284) -> ("file or folder exists?"=w283:bool, "dup path"=w281:path)  [unwired: 8 in, 1 out]
                n181 = case shown="真" w283 {
                  tunnel: [w296 w297] -> w282
                  tunnel: w281 -> [w295 w297]
                  tunnel: w280 -> [w294 _]
                  frame False {
                    n182 = Create Folder(prompt (Create Folder)=w294, path (use dialog)=w295) -> (created path=w296:path)  [unwired: 1 in, 2 out]
                  }
                  frame True {
                  }
                }
                n183 = Format Date/Time String(time format string (%c)="%y%m%d%H%M%S " ("时间格式字符串(%c)"), seconds (now)=w288) -> (date/time string=w276:string)  [unwired: 1 in]
                n184 = Path To String(path=w282) -> (string=w279:string)
                n185 = Concatenate Strings(w279, "\\" ("字符串")) -> (w277:string)
                n186 = Concatenate Strings(w277, w276) -> (w293:string)
                n187 = String To Path(string=w293) -> (path=→"最终存储路径":path)
              }
            }
          }
          frame True {
            n188 = local read "起始位置"() -> (w302:dbl[])
            n189 = local read "x轴终止位置"() -> (w313:dbl)
            n190 = local read "x轴起始位置"() -> (w312:dbl)
            n191 = local read "x轴步进长度"() -> (w310:dbl)
            n192 = local read "y轴终止位置"() -> (w307:sgl)
            n193 = local read "y轴起始位置"() -> (w306:sgl)
            n194 = local read "y轴步进长度"() -> (w305:sgl)
            n195 = call "Axis Group Move Relative.vi"("Target Displacement (units)"=w302, "error in (no error)"=w317, "Group Name (250 c max)"=w316, "connection ID in"=w318) -> ("error out"=w319:errorcluster, "connection ID out"=w320:T2)  [unwired: 5 in, 1 out]
            n196 = Subtract(x=w313, y=w312) -> (x-y=w311:dbl)
            n197 = Subtract(x=w307, y=w306) -> (x-y=w309:sgl)
            n198 = Divide(x=w309, y=w305) -> (x/y=w308:sgl)
            n199 = Divide(x=w311, y=w310) -> (x/y=→"X循环次数":dbl)
            n200 = Round To Nearest(number=w308) -> (nearest integer value=→"Y循环次数":sgl)
            n201 = call "XY Group Position Current Get.vi"("error in (no error)"=w319, "XY Group Name (250 c max)"=w316, "connection ID in"=w320) -> ("error out"=w303:errorcluster, "Current Position X & Y (units)"=w301:dbl[], "connection ID out"=w315:T2)  [unwired: 5 in, 1 out]
            n202 = local write "位置"(w301) -> ()
            n203 = stacked-sequence {
              tunnel: w316 -> [_ w332 _]
              tunnel: w315 -> [_ w331 _]
              tunnel: w303 -> [_ w327 _]
              tunnel: [_ w326 _] -> w300
              tunnel: [_ w325 _] -> w299
              tunnel: [_ w324 _] -> w298
              frame #0 {
                n204 = Wait (ms)(milliseconds to wait=u32 1000 ("等待时间（毫秒）")) -> ()  [unwired: 1 out]
              }
              frame #1 {
                n205 = local read "Y循环次数"() -> (w330:sgl)
                n206 = Add(x=w330, y=sgl 1.0) -> (x+y=w322:sgl)
                n207 = for {
                  N: w322 -> [_]
                  tunnel: w332 -> [w350]
                  tunnel: w331 -> [w351]
                  tunnel: [w344] -> w328 mode=indexing
                  tunnel: [w342] -> w323 mode=indexing
                  tunnel: w327 -> [w341]
                  tunnel: [w340] -> w326
                  tunnel: [w339] -> w325
                  tunnel: [w338] -> w324
                  tunnel: w322 -> [w335]
                  i -> [w349]
                  n208 = local read "X循环次数"() -> (w336:dbl)
                  n209 = Add(x=1, y=w349) -> (x+y=w347:i32)
                  n210 = Quotient & Remainder(x=w347, y=2) -> (floor(x/y)=w353:i32)  [unwired: 1 out]
                  n211 = Wait (ms)(milliseconds to wait=u32 3000 ("等待时间（毫秒）")) -> ()  [unwired: 1 out]
                  n212 = Add(x=w336, y=sgl 1.0) -> (x+y=w334:dbl)
                  n213 = Equal?(x=0, y=w353) -> (x = y?=w352:bool)
                  n214 = stacked-sequence {
                    tunnel: w352 -> [_ _ _ w452]
                    tunnel: w351 -> [_ w378 w444 w455]
                    tunnel: w350 -> [_ w377 w442 w454]
                    tunnel: [_ w368 _ _] -> w345
                    tunnel: [_ w376 _ _] -> w343
                    tunnel: [_ _ _ w452] -> w333
                    tunnel: w341 -> [_ w375 w443 _]
                    tunnel: [_ w374 _ _] -> w340
                    tunnel: [_ w373 _ _] -> w339
                    tunnel: [_ w372 _ _] -> w338
                    tunnel: w334 -> [_ w371 _ _]
                    tunnel: w335 -> [_ w370 _ _]
                    tunnel: w334 -> [_ w369 _ _]
                    frame #0 {
                      n215 = local read "y轴步进长度"() -> (w365:sgl)
                      n216 = local read "x轴步进长度"() -> (w362:dbl)
                      n217 = Build Array(0.0 ("元素"), w365) -> (w364:dbl[])
                      n218 = Build Array(w362, 0.0 ("元素")) -> (w367:dbl[])
                      n219 = local write "X移动量"(w367) -> ()
                      n220 = local write "Y移动量"(w364) -> ()
                    }
                    frame #1 {
                      n221 = for {
                        N: w371 -> [_]
                        tunnel: w377 -> [w428]
                        tunnel: w378 -> [w437]
                        tunnel: [w418] -> w376 mode=indexing
                        tunnel: w375 -> [w432]
                        tunnel: [w430] -> w374
                        tunnel: [w429] -> w373
                        tunnel: [w428] -> w372
                        tunnel: w370 -> [w427]
                        tunnel: w369 -> [w426]
                        tunnel: [w405] -> w368 mode=indexing
                        n222 = local read "计数器"() -> (w421:dbl)
                        n223 = call "Axis Group Move Relative.vi"("Target Displacement (units)"="X移动量", "error in (no error)"=w432, "Group Name (250 c max)"=w428, "connection ID in"=w437) -> ("error out"=w431:errorcluster, "connection ID out"=w436:T2)  [unwired: 5 in, 1 out]
                        n224 = Multiply(x=w427, y=w426) -> (x*y=w425:dbl)
                        n225 = Add(x=w421, y=1.0) -> (x+y=w419:dbl)
                        n226 = call "XY Group Position Current Get.vi"("error in (no error)"=w431, "XY Group Name (250 c max)"=w428, "connection ID in"=w436) -> ("error out"=w429:errorcluster, "Current Position X & Y (units)"=→"位置":dbl[], "connection ID out"=w430:T2)  [unwired: 5 in, 1 out]
                        n227 = local read "Area Number to Display"() -> (w411:i32)
                        n228 = local write "计数器"(w419) -> ()
                        n229 = local read "JYCCDLib.IJYCCDReqd"() -> (w416:refnum<k7>)
                        n230 = Divide(x=w419, y=w425) -> (x/y=w424:dbl)
                        n231 = Get Date/Time In Seconds() -> (seconds since 1Jan1904=w385:timestamp)
                        n232 = Multiply(x=w424, y=100.0) -> (x*y=→"采集进度":dbl)
                        n233 = local read "最终存储路径"() -> (w399:path)
                        n234 = Get Date/Time String(date format (0)=enum16{"short", "long", "abbreviated"}."abbreviated" ("日期格式(0)"), seconds (now)=w385, want seconds? (F)=TRUE ("需要秒？(F)")) -> (date string=w393:string, time string=w388:string)
                        n235 = local read "波长数组 2"() -> (w401:dbl[])
                        n236 = call "Convert to Dynamic Data2"("Array"=w401) -> ("Dynamic Data Type"=w404:dynamicdata)  [unwired: 3 in]
                        n237 = Search and Replace String(replace all?=TRUE ("替换全部？(F)"), input string=w388, search string=":" ("搜索字符串"), replace string="-" ("替换字符串(\"\")")) -> (result string=w392:string)  [unwired: 4 in, 3 out]
                        n238 = Path To String(path=w399) -> (string=w382:string)
                        n239 = call "MultiAccu - Acquire spectral.vi"("error in"=errorcluster {"status"=FALSE, "code"=0, "source"=""}, "Accumulations:"=u16 1, "ShutterOpen"=TRUE, "JYCCDLib.IJYCCDReqd"=w416) -> ("Acq Time(ms)"=w410:u32, "Array Out"=w412:i32[][][])  [unwired: 1 out]
                        n240 = Wait (ms)(milliseconds to wait=u32 3000 ("等待时间（毫秒）")) -> ()  [unwired: 1 out]
                        n241 = local write "Acq Time(ms)"(w410) -> ()
                        n242 = local read "Backlight"() -> (w408:i32[][])
                        n243 = Concatenate Strings(w382, w393, w392, "光谱" ("字符串"), ".xls" ("字符串")) -> (w397:string)
                        n244 = call "Array reset dimension.vi"("Area Number"=w411, "Array In"=w412) -> ("Array Out"=w409:i32[][])
                        n245 = String To Path(string=w397) -> (path=w398:path)
                        n246 = Subtract(x=w409, y=w408) -> (x-y=w407:i32[][])
                        n247 = Index Array(array=w407, index (row)=0 ("禁用的索引 (列)")) -> (element=w400:i32[])  [unwired: 1 in]
                        n248 = Reverse 1D Array(array=w400) -> (reversed array=w381:i32[])
                        n249 = call <vilib>:"Median Filter.vi"("left rank"=4, "X"=w381) -> ("Filtered X"=w380:dbl[])  [unwired: 8 in, 1 out]
                        n250 = call "Convert to Dynamic Data"("Array"=w380) -> ("Dynamic Data Type"=w402:dynamicdata)  [unwired: 3 in]
                        n251 = call "Build XY Graph"("Y Input"=w402, "X Input"=w404) -> ("XY Graph"=→"Spectrum":cluster{"Y":dbl[], "Y":dbl[]}[])  [unwired: 8 in, 1 out]
                        n252 = Array Max & Min(array=w380) -> (max value=w418:dbl, max index (indices)=w406:i32)  [unwired: 2 out]
                        "Intensity" <- w418
                        n253 = Index Array(array=w401, index=w406) -> (element=w405:dbl)
                        "POINT" <- w405
                        n254 = local write "Data"(w409) -> ()
                        n255 = local write "data 2"(w407) -> ()
                        n256 = call-poly <vilib>:"Write Delimited Spreadsheet.vi"("file path (dialog if empty)"=w398, "format (%.3f)"="%.16f", "1D data"=w380, "append to file? (new file:F)"=TRUE ("append to file? (F)"), "transpose? (no:F)"=TRUE ("transpose? (F)")) -> ()  [unwired: 9 in, 2 out]
                      }
                    }
                    frame #2 {
                      n257 = local read "X循环次数"() -> (w439:dbl)
                      n258 = local read "x轴步进长度"() -> (w450:dbl)
                      n259 = Add(x=w439, y=1.0) -> (x+y=w440:dbl)
                      n260 = Multiply(x=w450, y=w440) -> (x*y=w449:dbl)
                      n261 = Negate(x=w449) -> (-x=w448:dbl)
                      n262 = Build Array(w448, 0.0 ("元素")) -> (w445:dbl[])
                      n263 = call "Axis Group Move Relative.vi"("Target Displacement (units)"=w445, "error in (no error)"=w443, "Group Name (250 c max)"=w442, "connection ID in"=w444) -> ("connection ID out"=w446:T2)  [unwired: 5 in, 2 out]
                      n264 = call "XY Group Position Current Get.vi"("XY Group Name (250 c max)"=w442, "connection ID in"=w446) -> ()  [unwired: 6 in, 4 out]
                      n265 = Wait (ms)(milliseconds to wait=u32 200 ("等待时间（毫秒）")) -> ()  [unwired: 1 out]
                    }
                    frame #3 {
                      n266 = call "Axis Group Move Relative.vi"("Target Displacement (units)"="Y移动量", "Group Name (250 c max)"=w454, "connection ID in"=w455) -> ("connection ID out"=w456:T2)  [unwired: 6 in, 2 out]
                      n267 = call "XY Group Position Current Get.vi"("XY Group Name (250 c max)"=w454, "connection ID in"=w456) -> ()  [unwired: 6 in, 4 out]
                      n268 = Wait (ms)(milliseconds to wait=u32 200 ("等待时间（毫秒）")) -> ()  [unwired: 1 out]
                    }
                  }
                  n269 = case shown="假" w333 {
                    tunnel: w345 -> [w359 w361]
                    tunnel: [w358 w361] -> w344
                    tunnel: w343 -> [w357 w360]
                    tunnel: [w356 w360] -> w342
                    frame False {
                      n270 = Reverse 1D Array(array=w359) -> (reversed array=w358:dbl[])
                      n271 = Reverse 1D Array(array=w357) -> (reversed array=w356:dbl[])
                    }
                    frame True {
                    }
                  }
                }
                "波长数组" <- w328
                "强度数组" <- w323
              }
              frame #2 {
                n272 = local read "最终存储路径"() -> (w474:path)
                n273 = local read "最终存储路径"() -> (w493:path)
                n274 = Get Date/Time In Seconds() -> (seconds since 1Jan1904=w459:timestamp)
                n275 = Get Date/Time In Seconds() -> (seconds since 1Jan1904=w478:timestamp)
                n276 = Get Date/Time String(date format (0)=enum16{"short", "long", "abbreviated"}."abbreviated" ("日期格式(0)"), seconds (now)=w459, want seconds? (F)=TRUE ("需要秒？(F)")) -> (date string=w467:string, time string=w462:string)
                n277 = Get Date/Time String(date format (0)=enum16{"short", "long", "abbreviated"}."abbreviated" ("日期格式(0)"), seconds (now)=w478, want seconds? (F)=TRUE ("需要秒？(F)")) -> (date string=w486:string, time string=w481:string)
                n278 = Path To String(path=w474) -> (string=w475:string)
                n279 = Search and Replace String(replace all?=TRUE ("替换全部？(F)"), input string=w462, search string=":" ("搜索字符串"), replace string="-" ("替换字符串(\"\")")) -> (result string=w466:string)  [unwired: 4 in, 3 out]
                n280 = Path To String(path=w493) -> (string=w494:string)
                n281 = Search and Replace String(replace all?=TRUE ("替换全部？(F)"), input string=w481, search string=":" ("搜索字符串"), replace string="-" ("替换字符串(\"\")")) -> (result string=w485:string)  [unwired: 4 in, 3 out]
                n282 = local read "强度数组"() -> (w477:dbl[][])
                n283 = Concatenate Strings(w475, w467, w466, "波长.xls" ("字符串")) -> (w472:string)
                n284 = local read "波长数组"() -> (w458:dbl[][])
                n285 = Concatenate Strings(w494, w486, w485, "强度.xls" ("字符串")) -> (w491:string)
                n286 = String To Path(string=w472) -> (path=w473:path)
                n287 = String To Path(string=w491) -> (path=w492:path)
                n288 = call-poly <vilib>:"Write Delimited Spreadsheet.vi"("file path (dialog if empty)"=w473, "format (%.3f)"="%.16f", "2D data"=w458, "append to file? (new file:F)"=TRUE ("append to file? (F)"), "transpose? (no:F)"=TRUE ("transpose? (F)")) -> ()  [unwired: 9 in, 2 out]
                n289 = call-poly <vilib>:"Write Delimited Spreadsheet.vi"("file path (dialog if empty)"=w492, "format (%.3f)"="%.16f", "2D data"=w477, "append to file? (new file:F)"=TRUE ("append to file? (F)"), "transpose? (no:F)"=TRUE ("transpose? (F)")) -> ()  [unwired: 9 in, 2 out]
                n290 = call-poly <vilib>:"Plot Helper.vi"("z matrix"=w458) -> ("3D Plot lvclass Array out"=→"波长3维图":refnum<class "3D Plot Datatype.lvclass">[])  [unwired: 5 in, 5 out]
                n291 = call-poly <vilib>:"Plot Helper.vi"("z matrix"=w477) -> ("3D Plot lvclass Array out"=→"强度三维图":refnum<class "3D Plot Datatype.lvclass">[])  [unwired: 5 in, 5 out]
              }
            }
          }
        }
      }
    }
    n292 = local write "计数器"(0.0 ("计数器")) -> ()
    n293 = local write "强度数组"(w201) -> ()
    n294 = local write "波长数组"(w201) -> ()
    n295 = local read "Close"() -> (w193:bool)
  }
  n296 = stacked-sequence {
    seq-local: [_ _ w504 _ _] -> [_ _ _ w514 w519]
    seq-local: [_ _ w503 _ _] -> [_ _ _ w513 _]
    seq-local: [_ _ _ w512 _] -> [_ _ _ _ _]
    frame #0 {
      n297 = call "Get Monos From Config Browser.vi"() -> ("UniqueIDs"=w499:string[], "Mono ID"=w500:string[])  [unwired: 3 in, 1 out]
      n298 = Build Cluster Array(w500, w499) -> (w497:cluster{"String":string, "String":string}[])
      n299 = property on="Mono ID" class="CmbBox"("Strings And Values []"=w497) -> ()  [unwired: 2 in, 2 out]
      n300 = Index Array(array=w497, index=0) -> (element=w498:cluster{"String":string, "String":string})
      n301 = Unbundle(w498) -> ("String"=w495:string)  [unwired: 1 out]
      "Current UniqueID" <- w495
      n302 = local write "Mono ID"(w495) -> ()
    }
    frame #1 {
      n303 = while {
        stop <- "Connect" stop-if-true
        n304 = local read "Mono ID"() -> (w501:string)
        n305 = local write "Current UniqueID"(w501) -> ()
      }
    }
    frame #2 {
      n306 = local read "Mono ID"() -> (w506:string)
      n307 = call "JYInitMono.vi"("Unique ID"=w506, "Force Init"="Force\nInitialization") -> ("Refnum out"=w504:refnum<k7>, "Initialized"=→"Initialized JY":bool, "error out"=w503:errorcluster)  [unwired: 9 in, 2 out]
    }
    frame #3 {
      n308 = call "Show Current Grating.vi"("Refnum in"=w514, "error in (no error)"=w513) -> ("Gratings"=w515:dbl[], "Grating Index"=w509:i32, "Current Grating"=w511:dbl, "Current Description"=w508:string, "error out"=w512:errorcluster)  [unwired: 5 in, 4 out]
      "Gratings" <- w515
      n309 = local write "Current Grating"(w511) -> ()
      n310 = local write "Current Description"(w508) -> ()
      n311 = Number To Decimal String(number=w515) -> (decimal integer string=w517:string[])  [unwired: 1 in]
      n312 = Number To Decimal String(number=w509) -> (decimal integer string=w510:string)  [unwired: 1 in]
      n313 = property on="Target Grating" class="CmbBox"("Value"=w510) -> ()  [unwired: 2 in, 2 out]
      n314 = Build Cluster Array(w517, string[] ["1", "2", "3"]) -> (w518:cluster{"Numeric":string, string}[])
      n315 = property on="Target Grating" class="CmbBox"("Strings And Values []"=w518) -> ()  [unwired: 2 in, 2 out]
    }
    frame #4 {
      n316 = while {
        tunnel: w519 -> [w521]
        stop <- w520 stop-if-true
        n317 = stacked-sequence {
          seq-local: [w525 _ _ _ _] -> [_ w532 w543 _ w550]
          seq-local: [w524 _ _ _ _] -> [_ w531 w542 _ _]
          seq-local: [_ w530 _ _ _] -> [_ _ _ _ _]
          seq-local: [_ w529 _ _ _] -> [_ _ _ _ _]
          seq-local: [_ _ w535 _ _] -> [_ _ _ _ _]
          seq-local: [_ _ w534 _ _] -> [_ _ _ w545 _]
          tunnel: w521 -> [w523 _ _ w546 _]
          frame #0 {
            n318 = call "Show Current Grating.vi"("Refnum in"=w523) -> ("Grating Index"=→"Grating Index":i32, "Current Grating"=→"Current Grating":dbl, "Current Description"=→"Current Description":string, "error out"=w524:errorcluster, "JYMONOLib.IJYMonoReqd"=w525:refnum<k7>)  [unwired: 6 in, 4 out]
          }
          frame #1 {
            n319 = call "JYGetCurrentWL.vi"("error in (no error)"=w531, "JYMONOLib.IJYMonoReqd"=w532) -> ("error out"=w529:errorcluster, "Units"=→"Units":string, "Current WL"=→"Current WL":dbl, "JYMONOLib.IJYMonoReqd 2"=w530:refnum<k7>)  [unwired: 6 in]
          }
          frame #2 {
            w540 = u16 1 items=["Entrance", "Exit"] ("Mirror Number")
            w541 = u16 0 items=["Entrance", "Exit"] ("Mirror Number")
            n320 = call "JYGetMirrorPos.vi"("error in (no error)"=w542, "Mirror"=w541, "Refnum In"=w543) -> ("error out"=w538:errorcluster, "Current Mirror Position"=→"Entrance Mirror\nPosition":i32, "Refnum Out"=w539:refnum<k7>)  [unwired: 1 in]
            n321 = call "JYGetMirrorPos.vi"("error in (no error)"=w538, "Mirror"=w540, "Refnum In"=w539) -> ("error out"=w534:errorcluster, "Current Mirror Position"=→"Exit Mirror\nPosition":i32, "Refnum Out"=w535:refnum<k7>)  [unwired: 1 in]
          }
          frame #3 {
            w548 = u16 0 items=["Front Entrance", "Side Entrance", "Front Exit", "Side Exit", "First Intermediate", "Second Intermediate"] ("Slit")
            n322 = call "JYGetSlits.vi"("MonoRefNum IN"=w546, "Slit"=w548, "error in (no error)"=w545) -> ("Units"=→"Units 2":string, "Slit Width"=→"Front Entrance":dbl, "error out"=→"error out":errorcluster)  [unwired: 13 in, 1 out]
          }
          frame #4 {
            n323 = local read "Move To\nTarget Positions"() -> (w551:bool)
            n324 = case shown="真" w551 {
              tunnel: w550 -> [_ w552]
              frame False {
              }
              frame True {
                n325 = stacked-sequence {
                  seq-local: [w554 _ _ _] -> [_ w560 _ _]
                  seq-local: [_ w558 _ _] -> [_ _ w575 _]
                  seq-local: [_ _ w562 _] -> [_ _ _ w581]
                  seq-local: [_ _ _ w578] -> [_ _ _ _]
                  tunnel: w552 -> [w556 w559 w573 w582]
                  frame #0 {
                    n326 = property on="Target Grating" class="CmbBox"() -> ("Value"=w553:string)  [unwired: 2 in, 2 out]
                    n327 = local read "error out"() -> (w555:errorcluster)
                    n328 = Decimal String To Number(string=w553) -> (number=w557:i32)  [unwired: 2 in, 1 out]
                    n329 = call "JYTurret.vi"("error in (no error)"=w555, "Grating Index"=w557, "JYMONOLib.IJYMonoReqd"=w556) -> ("error out"=w554:errorcluster)  [unwired: 2 out]
                  }
                  frame #1 {
                    # "Move Grating to Target Position"
                    n330 = call "JYMoveToWavelength.vi"("error in (no error)"=w560, "Target WL"="Target WL", "RefNum In"=w559) -> ("error out"=w558:errorcluster)  [unwired: 1 in, 2 out]
                  }
                  frame #2 {
                    w568 = u16 1 items=["Entrance", "Exit"] ("Mirror Number")
                    w567 = u16 0 items=["Entrance", "Exit"] ("Mirror Number")
                    w574 = u16 1 items=["Entrance", "Exit", "Front", "Side"] ("Mirror Number")
                    w577 = u16 0 items=["Entrance", "Exit", "Front", "Side"] ("Mirror Number")
                    # "Move Mirrors"
                    n331 = call "JYMirrorMove.vi"("error in (no error)"=w575, "Mirror Position"="Entrance Mirror", "Mirror Number"=w577, "RefNum In"=w573) -> ("error out"=w572:errorcluster)  [unwired: 6 in, 1 out]
                    n332 = call "JYMirrorMove.vi"("error in (no error)"=w572, "Mirror Position"="Exit Mirror", "Mirror Number"=w574, "RefNum In"=w573) -> ("error out"=w565:errorcluster, "MonoRefNum Out"=w566:refnum<k7>)  [unwired: 6 in]
                    n333 = call "JYGetMirrorPos.vi"("error in (no error)"=w565, "Mirror"=w567, "Refnum In"=w566) -> ("error out"=w570:errorcluster, "Current Mirror Position"=w564:i32, "Refnum Out"=w569:refnum<k7>)  [unwired: 1 in]
                    n334 = local write "Entrance Mirror\nPosition"(w564) -> ()
                    n335 = call "JYGetMirrorPos.vi"("error in (no error)"=w570, "Mirror"=w568, "Refnum In"=w569) -> ("error out"=w562:errorcluster, "Current Mirror Position"=w563:i32)  [unwired: 1 in, 1 out]
                    n336 = local write "Exit Mirror\nPosition"(w563) -> ()
                  }
                  frame #3 {
                    w580 = u16 0 items=["Front Entrance", "Side Entrance", "Front Exit", "Side Exit", "First Intermediate", "Second Intermediate"] ("Slit")
                    # "Set New Slit Positions"
                    n337 = call "JYSlits.vi"("JYMONOLib.IJYMonoReqd"=w582, "Slit"=w580, "error in (no error)"=w581, "Slit Width"="Target\nFront Entrance") -> ("error out"=w578:errorcluster)  [unwired: 1 in, 1 out]
                  }
                }
              }
            }
          }
        }
        n338 = local read "Close"() -> (w520:bool)
      }
    }
  }
  n339 = call "Group Kill.vi"("error in (no error)"=w6, "Group Name (250 c max)"=w5, "connection ID in"=w7) -> ("error out"=w8:errorcluster, "connection ID out"=w9:T2)  [unwired: 6 in, 1 out]
  n340 = call "Close TCP-IP.vi"("error in (no error)"=w8, "connection ID in"=w9) -> ()  [unwired: 9 in, 1 out]
  "Backlight" <- i32[][] [] ("Backlight")
  "data 2" <- i32[][] [] ("data 2")
